vi "Persistence.vi"() -> ()   [LabVIEW 2020]
uses:
  ColorSelection.ctl
  d94e0766-a9f8-4b91-b199-a4dd9911b6b9.vi
  <vilib>/measure/NI_MABase.lvlib
panel:
  in  "Color 2":T1
  in  "Color 1":T1=enum."Green"
  out "Palette 2":u32[](array[colorbox])=[16711680, 16715535, 16719390, 16723245, 16727100, 16730955, 16734810, 16738665, 16742520, 16746375, 16750230, 16754085, 16757940, 16761795, 16765650, 16769505, 16773360]
  in  "Signal Type 2":enum16{"Sine", "Gauss", "Sine + Gauss"}(ring)=enum."Sine + Gauss"
  out "Buffer Depth 2":i32=17
  out "Buffer Depth 1":i32=17
  in  "Combine signals to Signal 2":enum16{"None", "Add 1 and 2"}(ring)
  in  "Signal Type 1":enum16{"Sine", "Gauss", "Sine + Gauss"}(ring)=enum."Sine + Gauss"
  in  "frequency 2":dbl=3.0 format="%0.2p"
  in  "amplitude 2":dbl=0.75 format="%0.2p"
  in  "phase 2 [deg]":dbl=-2.0
  in  "sampling info 2":cluster{"Fs":dbl, "#s":dbl}={"Fs"=1000.0, "#s"=1000.0} {"Fs" format="%.2p"}
  out "Palette 1":u32[](array[colorbox])=[65280, 1048335, 2031390, 3014445, 3997500, 4980555, 5963610, 6946665, 7929720, 8912775, 9895830, 10878885, 11861940, 12844995, 13828050, 14811105, 15794160]
  in  "Persistence Depth":u32=17
  out "Combined Plots":waveform(dbl)[](graph)=[{"t0"=timestamp(0 s since 1904-01-01), "dt"=0.001, "Y"=array[1000 elements]}, {"t0"=timestamp(0 s since 1904-01-01), "dt"=0.001, "Y"=array[1000 elements]}, {"t0"=timestamp(0 s since 1904-01-01), "dt"=0.001, "Y"=array[1000 elements]}, {"t0"=timestamp(0 s since 1904-01-01), "dt"=0.001, "Y"=array[1000 elements]}, {"t0"=timestamp(0 s since 1904-01-01), "dt"=0.001, "Y"=array[1000 elements]}, {"t0"=timestamp(0 s since 1904-01-01), "dt"=0.001, "Y"=array[1000 elements]}, {"t0"=timestamp(0 s since 1904-01-01), "dt"=0.001, "Y"=array[1000 elements]}, {"t0"=timestamp(0 s since 1904-01-01), "dt"=0.001, "Y"=array[1000 elements]}, {"t0"=timestamp(0 s since 1904-01-01), "dt"=0.001, "Y"=array[1000 elements]}, {"t0"=timestamp(0 s since 1904-01-01), "dt"=0.001, "Y"=array[1000 elements]}, {"t0"=timestamp(0 s since 1904-01-01), "dt"=0.001, "Y"=array[1000 elements]}, {"t0"=timestamp(0 s since 1904-01-01), "dt"=0.001, "Y"=array[1000 elements]}, {"t0"=timestamp(0 s since 1904-01-01), "dt"=0.001, "Y"=array[1000 elements]}, {"t0"=timestamp(0 s since 1904-01-01), "dt"=0.001, "Y"=array[1000 elements]}, {"t0"=timestamp(0 s since 1904-01-01), "dt"=0.001, "Y"=array[1000 elements]}, {"t0"=timestamp(0 s since 1904-01-01), "dt"=0.001, "Y"=array[1000 elements]}, {"t0"=timestamp(0 s since 1904-01-01), "dt"=0.001, "Y"=array[1000 elements]}, {"t0"=timestamp(0 s since 1904-01-01), "dt"=0.001, "Y"=array[1000 elements]}, {"t0"=timestamp(0 s since 1904-01-01), "dt"=0.001, "Y"=array[1000 elements]}, {"t0"=timestamp(0 s since 1904-01-01), "dt"=0.001, "Y"=array[1000 elements]}, {"t0"=timestamp(0 s since 1904-01-01), "dt"=0.001, "Y"=array[1000 elements]}, {"t0"=timestamp(0 s since 1904-01-01), "dt"=0.001, "Y"=array[1000 elements]}, {"t0"=timestamp(0 s since 1904-01-01), "dt"=0.001, "Y"=array[1000 elements]}, {"t0"=timestamp(0 s since 1904-01-01), "dt"=0.001, "Y"=array[1000 elements]}, {"t0"=timestamp(0 s since 1904-01-01), "dt"=0.001, "Y"=array[1000 elements]}, {"t0"=timestamp(0 s since 1904-01-01), "dt"=0.001, "Y"=array[1000 elements]}, {"t0"=timestamp(0 s since 1904-01-01), "dt"=0.001, "Y"=array[1000 elements]}, {"t0"=timestamp(0 s since 1904-01-01), "dt"=0.001, "Y"=array[1000 elements]}, {"t0"=timestamp(0 s since 1904-01-01), "dt"=0.001, "Y"=array[1000 elements]}, {"t0"=timestamp(0 s since 1904-01-01), "dt"=0.001, "Y"=array[1000 elements]}, {"t0"=timestamp(0 s since 1904-01-01), "dt"=0.001, "Y"=array[1000 elements]}, {"t0"=timestamp(0 s since 1904-01-01), "dt"=0.001, "Y"=array[1000 elements]}, {"t0"=timestamp(0 s since 1904-01-01), "dt"=0.001, "Y"=array[1000 elements]}, {"t0"=timestamp(0 s since 1904-01-01), "dt"=0.001, "Y"=array[1000 elements]}]
  in  "frequency":dbl=10.0 format="%0.2p"
  in  "amplitude":dbl=1.0 format="%0.2p"
  in  "phase [deg]":dbl=3.0
  in  "sampling info":cluster{"Fs":dbl, "#s":dbl}={"Fs"=1000.0, "#s"=1000.0} {"Fs" format="%.2p"}
  in  "stop":bool
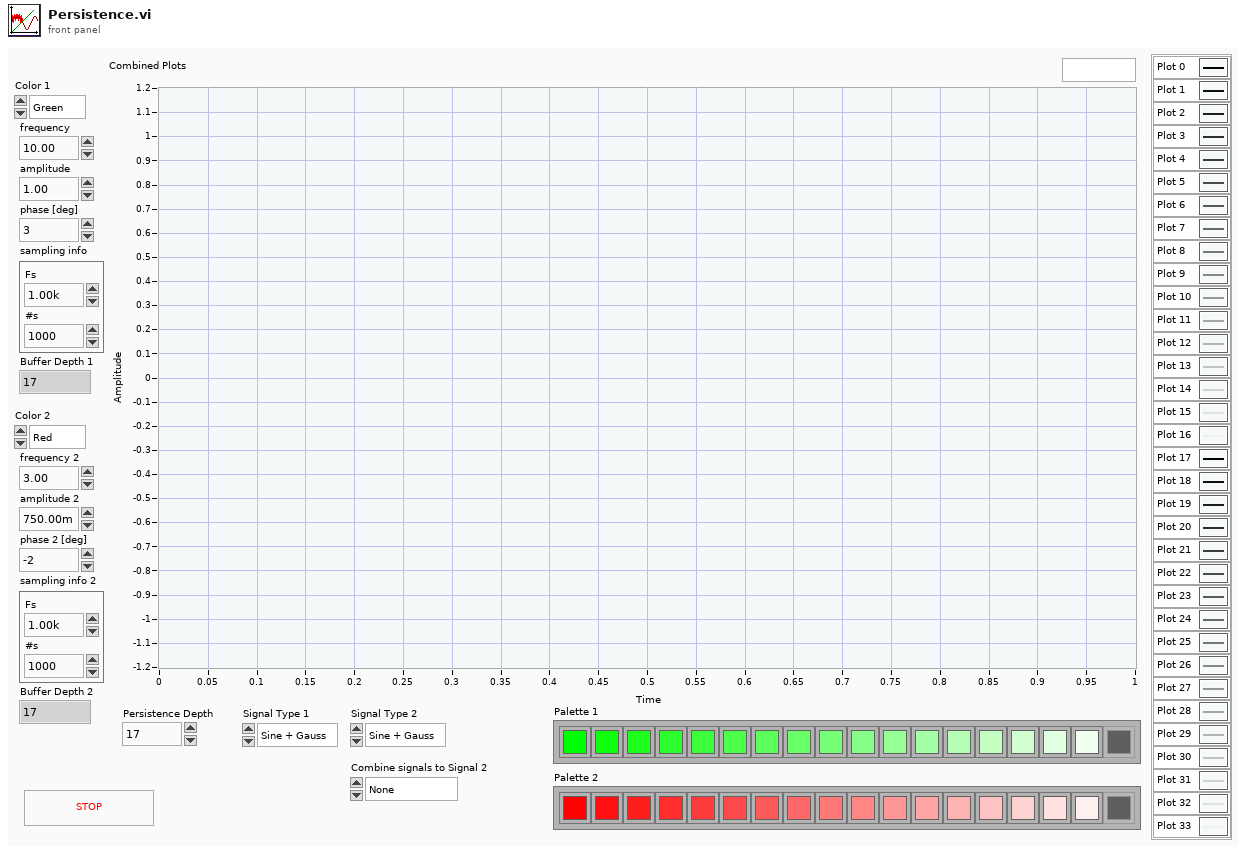
[diagram p1: front panel]
types:
  T1 = typedef "ColorSelection.ctl" = enum16{"Red", "Green", "Blue", "Yellow", "Magenta", "Cyan", "White", "Black"}
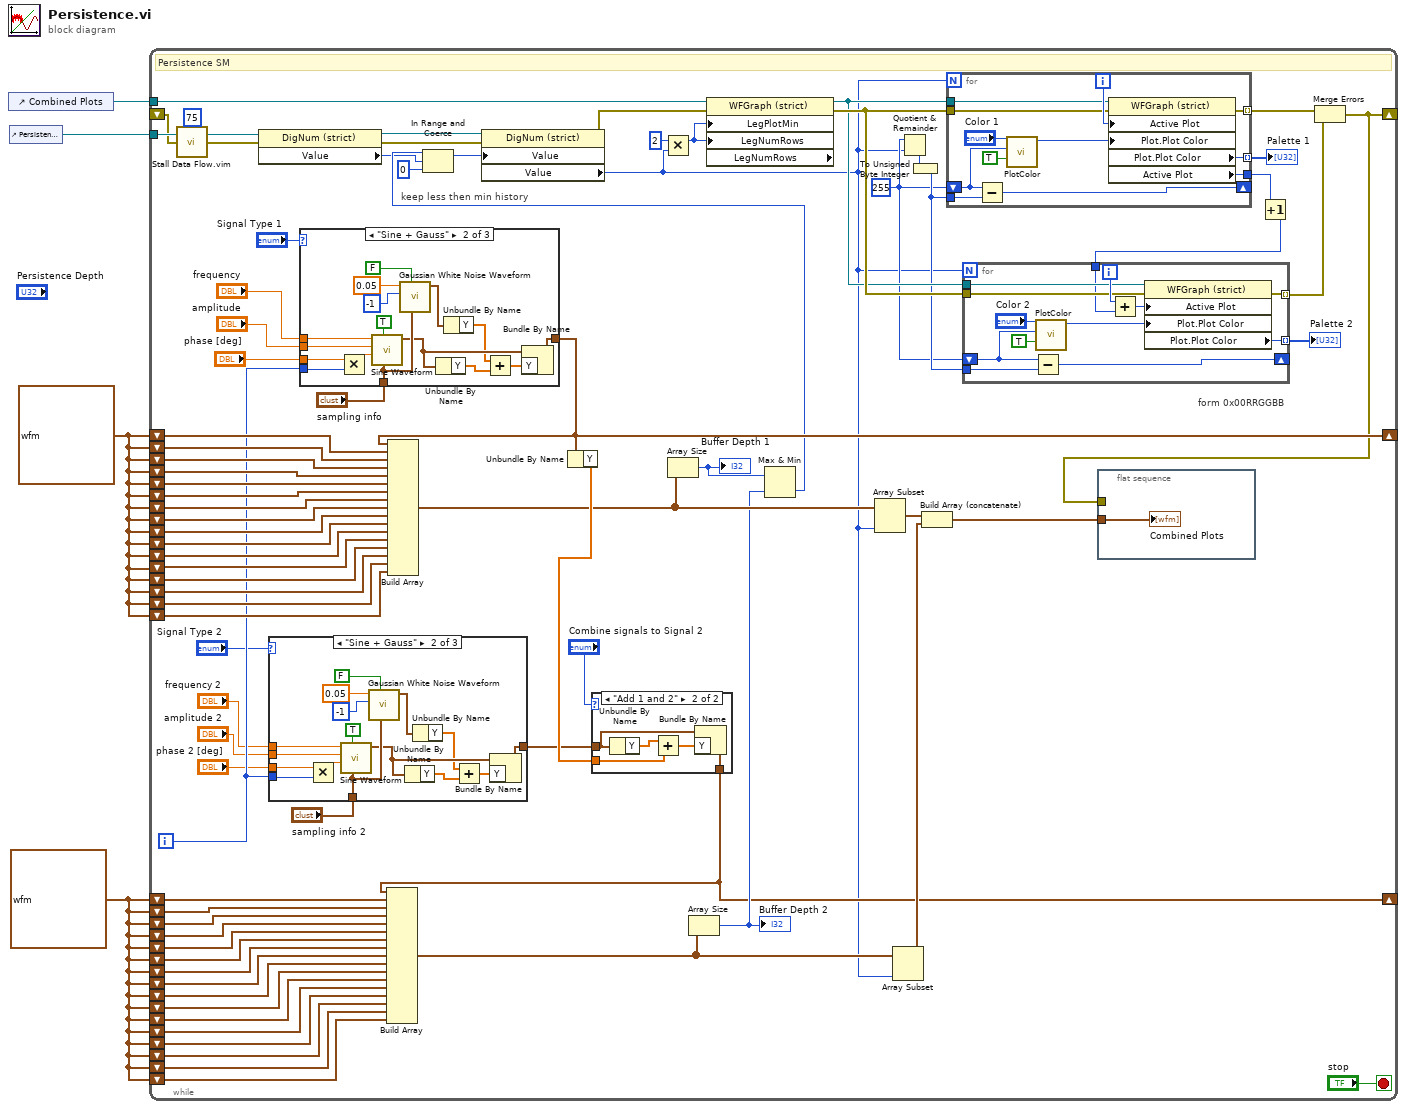
[diagram p0: block diagram]
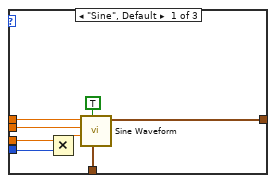
[diagram p2: hidden frame]
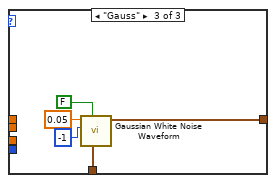
[diagram p3: hidden frame]
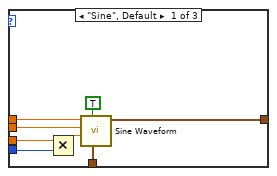
[diagram p5: hidden frame]
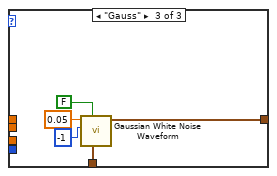
[diagram p6: hidden frame]
diagram:
  w4 = waveform(dbl) {"t0"=timestamp(0 s since 1904-01-01), "dt"=1.0, "Y"=[]} ("signal out")
  w3 = waveform(dbl) {"t0"=timestamp(0 s since 1904-01-01), "dt"=1.0, "Y"=[]} ("signal out")
  n1 = control-ref of="Combined Plots"() -> (w2:refnum<vi>)
  n2 = control-ref of="Persistence Depth"() -> (w1:refnum<vi>)
  n3 = while {
    shift-right: [w46] -> _
    shift-left: w3 -> [w76]
    shift-left: w3 -> [w85]
    shift-left: w3 -> [w84]
    shift-left: w3 -> [w83]
    shift-left: w3 -> [w82]
    shift-left: w3 -> [w81]
    shift-left: w3 -> [w80]
    shift-left: w3 -> [w79]
    shift-left: w3 -> [w78]
    shift-left: w3 -> [w77]
    shift-left: w3 -> [w75]
    shift-left: w3 -> [w74]
    shift-right: [w27] -> _
    shift-left: w4 -> [w70]
    shift-left: w4 -> [w69]
    shift-left: w4 -> [w68]
    shift-left: w4 -> [w67]
    shift-left: w4 -> [w66]
    shift-left: w4 -> [w65]
    shift-left: w4 -> [w64]
    shift-left: w4 -> [w63]
    shift-left: w4 -> [w62]
    shift-left: w4 -> [w61]
    shift-left: w4 -> [w60]
    shift-left: w4 -> [w59]
    shift-left: w4 -> [w58]
    shift-left: w4 -> [w57]
    shift-left: w3 -> [w43]
    shift-left: w3 -> [w42]
    shift-left: w3 -> [w41]
    shift-left: w4 -> [w30]
    shift-left: w4 -> [w29]
    shift-left: w3 -> [w28]
    tunnel: w2 -> [w26]
    tunnel: w1 -> [w25]
    shift-right: [w5] -> _
    shift-left: _ -> [w8]
    i -> [w16]
    stop <- "stop" stop-if-true
    w52 = u8 255
    # "keep less then min history"
    # "form 0x00RRGGBB"
    # "Persistence SM"
    n4 = call "Stall Data Flow.vim"("value in"=w8, "milliseconds to wait"=u32 75) -> ("value out"=w7:errorcluster)  [unwired: 1 out]
    n5 = property class="DigNum (strict)"(reference=w25, error in=w7) -> (reference out=w32:refnum<vi>, error out=w24:errorcluster, "Value"=w33:u32)
    n6 = case shown="\"Sine + Gauss\"" "Signal Type 2" {
      tunnel: "sampling info 2" -> [w90 w103 w113]
      tunnel: w16 -> [w94 w110 _]
      tunnel: [w89 w99 w114] -> w18
      tunnel: "phase 2 [deg]" -> [w93 w109 _]
      tunnel: "amplitude 2" -> [w92 w108 _]
      tunnel: "frequency 2" -> [w91 w107 _]
      frame "Sine", Default {
        n7 = Multiply(x=w93, y=w94) -> (x*y=w95:dbl)
        n8 = call <vilib>:"Sine Waveform.vi"("sampling info"=w90, "reset signal"=TRUE, "phase"=w95, "amplitude"=w92, "frequency"=w91) -> ("signal out"=w89:waveform(dbl))  [unwired: 5 in, 1 out]
      }
      frame "Sine + Gauss" {
        n9 = Multiply(x=w109, y=w110) -> (x*y=w111:dbl)
        n10 = call <vilib>:"Sine Waveform.vi"("sampling info"=w103, "reset signal"=TRUE, "phase"=w111, "amplitude"=w108, "frequency"=w107) -> ("signal out"=w100:waveform(dbl))  [unwired: 5 in, 1 out]
        n11 = call <vilib>:"Gaussian White Noise Waveform.vi"("sampling info"=w103, "reset signal"=FALSE, "seed"=-1, "standard deviation"=0.05) -> ("signal out"=w98:waveform(dbl))  [unwired: 6 in, 1 out]
        n12 = Unbundle By Name(w100) -> ("Y"=w102:dbl[])
        n13 = Unbundle By Name(w98) -> ("Y"=w97:dbl[])
        n14 = Add(x=w97, y=w102) -> (x+y=w101:dbl[])
        n15 = Bundle By Name(cluster=w100, "Y"=w101) -> (w99:waveform(dbl))
      }
      frame "Gauss" {
        n16 = call <vilib>:"Gaussian White Noise Waveform.vi"("sampling info"=w113, "reset signal"=FALSE, "seed"=-1, "standard deviation"=0.05) -> ("signal out"=w114:waveform(dbl))  [unwired: 6 in, 1 out]
      }
    }
    n17 = case shown="\"Sine + Gauss\"" "Signal Type 1" {
      tunnel: "sampling info" -> [w125 w138 w148]
      tunnel: w16 -> [w129 w145 _]
      tunnel: [w124 w134 w149] -> w46
      tunnel: "phase [deg]" -> [w128 w144 _]
      tunnel: "amplitude" -> [w127 w143 _]
      tunnel: "frequency" -> [w126 w142 _]
      frame "Sine", Default {
        n18 = Multiply(x=w128, y=w129) -> (x*y=w130:dbl)
        n19 = call <vilib>:"Sine Waveform.vi"("sampling info"=w125, "reset signal"=TRUE, "phase"=w130, "amplitude"=w127, "frequency"=w126) -> ("signal out"=w124:waveform(dbl))  [unwired: 5 in, 1 out]
      }
      frame "Sine + Gauss" {
        n20 = Multiply(x=w144, y=w145) -> (x*y=w146:dbl)
        n21 = call <vilib>:"Sine Waveform.vi"("sampling info"=w138, "reset signal"=TRUE, "phase"=w146, "amplitude"=w143, "frequency"=w142) -> ("signal out"=w135:waveform(dbl))  [unwired: 5 in, 1 out]
        n22 = call <vilib>:"Gaussian White Noise Waveform.vi"("sampling info"=w138, "reset signal"=FALSE, "seed"=-1, "standard deviation"=0.05) -> ("signal out"=w133:waveform(dbl))  [unwired: 6 in, 1 out]
        n23 = Unbundle By Name(w135) -> ("Y"=w137:dbl[])
        n24 = Unbundle By Name(w133) -> ("Y"=w132:dbl[])
        n25 = Add(x=w132, y=w137) -> (x+y=w136:dbl[])
        n26 = Bundle By Name(cluster=w135, "Y"=w136) -> (w134:waveform(dbl))
      }
      frame "Gauss" {
        n27 = call <vilib>:"Gaussian White Noise Waveform.vi"("sampling info"=w148, "reset signal"=FALSE, "seed"=-1, "standard deviation"=0.05) -> ("signal out"=w149:waveform(dbl))  [unwired: 6 in, 1 out]
      }
    }
    n28 = Build Array(w46, w76, w85, w84, w83, w82, w81, w80, w79, w78, w77, w75, w74, w43, w42, w41, w28) -> (w40:waveform(dbl)[])
    n29 = Unbundle By Name(w46) -> ("Y"=w45:dbl[])
    n30 = case shown="\"Add 1 and 2\"" "Combine signals to Signal 2" {
      tunnel: w18 -> [w118 w122]
      tunnel: [w118 w121] -> w27
      tunnel: w45 -> [_ w119]
      frame "None", Default {
      }
      frame "Add 1 and 2" {
        n31 = Unbundle By Name(w122) -> ("Y"=w123:dbl[])
        n32 = Add(x=w123, y=w119) -> (x+y=w120:dbl[])
        n33 = Bundle By Name(cluster=w122, "Y"=w120) -> (w121:waveform(dbl))
      }
    }
    n34 = Build Array(w27, w70, w69, w68, w67, w66, w65, w64, w63, w62, w61, w60, w59, w58, w57, w30, w29) -> (w38:waveform(dbl)[])
    n35 = Array Size(array=w40) -> (size(s)=w37:i32)
    "Buffer Depth 1" <- w37
    n36 = Array Size(array=w38) -> (size(s)=w36:i32)
    "Buffer Depth 2" <- w36
    n37 = Max & Min(x=w37, y=w36) -> (min(x,y)=w35:i32)  [unwired: 1 out]
    n38 = In Range and Coerce(upper limit=w35, x=w33, lower limit=u32 0) -> (coerced(x)=w31:u32)  [unwired: 1 out]
    n39 = property class="DigNum (strict)"(reference=w32, error in=w24, "Value"=w31) -> (error out=w23:errorcluster, "Value"=w22:u32)  [unwired: 1 out]
    n40 = Multiply(x=u32 2 ("y"), y=w22) -> (x*y=w50:u32)
    n41 = property on="Property Node" class="WFGraph (strict)" props=["LegPlotMin", "LegNumRows", "LegNumRows"](reference=w26, error in=w23, "LegPlotMin"=w50, "LegNumRows"=w50) -> (reference out=w54:refnum<vi>, error out=w55:errorcluster)  [unwired: 1 out]
    n42 = Array Subset(array=w40, length=w22) -> (w72:waveform(dbl)[])  [unwired: 1 in]
    n43 = Array Subset(array=w38, length=w22) -> (w39:waveform(dbl)[])  [unwired: 1 in]
    n44 = Quotient & Remainder(x=w52, y=w22) -> (floor(x/y)=w73:u32)  [unwired: 1 out]
    n45 = To Unsigned Byte Integer(number=w73) -> (unsigned 8bit integer=w53:u8)
    n46 = Build Array (concatenate)(w72, w39) -> (w56:waveform(dbl)[])
    n47 = for {
      N: w22 -> [_]
      shift-right: [w174] -> _
      shift-left: w52 -> [w168]
      tunnel: w53 -> [w175]
      tunnel: w54 -> [w173]
      tunnel: w55 -> [w172]
      tunnel: [w171] -> w71 mode=indexing
      tunnel: [w170] -> w51
      tunnel: [w169] -> w10 mode=indexing
      i -> [w177]
      n48 = Subtract(x=w168, y=w175) -> (x-y=w174:u8)
      n49 = call "PlotColor.vi"("White Palette"=TRUE, "InputColorCode"=w168, "Color"="Color 1") -> ("Color"=w176:u32)  [unwired: 8 in]
      n50 = property on="Property Node" class="WFGraph (strict)"(reference=w173, error in=w172, "Active Plot"=w177, "Plot.Plot Color"=w176) -> (error out=w169:errorcluster, "Plot.Plot Color"=w171:u32, "Active Plot"=w170:u32)  [unwired: 1 out]
    }
    "Palette 1" <- w71
    n51 = flat-sequence {
      tunnel: w56 -> [w88]
      tunnel: w5 -> [_]
      frame #0 {
        "Combined Plots" <- w88
      }
    }
    n52 = Increment(x=w51) -> (x+1=w48:u32)
    n53 = for {
      N: w22 -> [_]
      shift-right: [w163] -> _
      shift-left: w52 -> [w154]
      tunnel: w53 -> [w164]
      tunnel: w54 -> [w162]
      tunnel: w55 -> [w161]
      tunnel: [w160] -> w11 mode=indexing
      tunnel: w48 -> [w158]
      tunnel: [w157] -> w9 mode=indexing
      i -> [w165]
      n54 = Subtract(x=w154, y=w164) -> (x-y=w163:u8)
      n55 = call "PlotColor.vi"("White Palette"=TRUE, "InputColorCode"=w154, "Color"="Color 2") -> ("Color"=w153:u32)  [unwired: 8 in]
      n56 = Add(x=w165, y=w158) -> (x+y=w159:u32)
      n57 = property on="Property Node" class="WFGraph (strict)"(reference=w162, error in=w161, "Active Plot"=w159, "Plot.Plot Color"=w153) -> (error out=w157:errorcluster, "Plot.Plot Color"=w160:u32)  [unwired: 1 out]
    }
    "Palette 2" <- w11
    n58 = Merge Errors(w10, w9) -> (w5:errorcluster)
  }
